vi "Add content to Engine library.vi"(6 "Project Name":string, 8 "error in":errorcluster, 9 "Project Root":path, 10 "CD Wizard - Internal Data":T1, 11 "CD Template":refnum<class "NIVS_PPL_Inline HW Interface.lvclass">) -> (0 "error out":errorcluster)   [LabVIEW 2020, in "NIVS_PPL_Inline HW Interface.lvclass"]
doc: "Add all virtual folders and VIs to the Engine library."
uses:
  NIVS_PPL_Inline HW Interface.lvclass
  NIVS_Consolidated_CDW_MetaDataObj/Internal data.ctl
  C:/dev/Karthick/FPGA Addons Packages/niveristand-custom-device-wizard/ProjectTemplate/Source/NI VeriStand/Custom Device/Template Classes/NIVS_CD Template/NIVS_CD Template.lvclass
  NIVS_Consolidated_CDW_MetaDataObj/CD Engine lvlib.ctl
  NIVS_Consolidated_CDW_MetaDataObj/Add Item - Type.ctl
  NIVS_CD Template/NIVS_CD Template.lvclass/NIVS_CD Template.ctl
  NIVS_Consolidated_CDW_MetaDataObj/CD Engine lvlib.vi
  NIVS_Consolidated_CDW_MetaDataObj/NIVS_Consolidated_CDW_MetaDataObj.lvclass
  NIVS_CD Template/NIVS_CD Template.lvclass
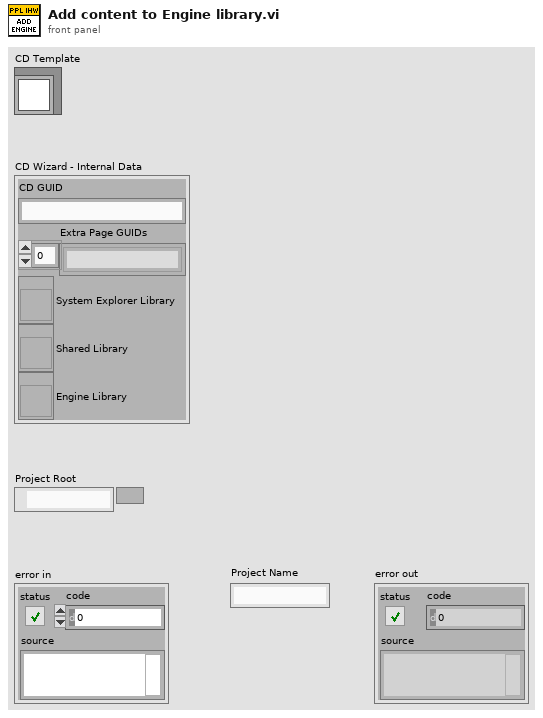
[diagram p1: front panel]
types:
  T1 = typedef "NIVS_Consolidated_CDW_MetaDataObj.lvclass/Internal data.ctl" = cluster{"CD GUID":string, "Extra Page GUIDs":string[], "System Explorer Library":refnum<vi>, "Shared Library":refnum<vi>, "Engine Library":refnum<vi>}
  T2 = typedef "NIVS_Consolidated_CDW_MetaDataObj.lvclass/CD Engine lvlib.ctl" = enum16{"LibraryFileName", "LibraryFolderName", "Engine.FolderName", "Engine.Init.FolderName", "Engine.Run.FolderName", "Engine.Shutdown.FolderName", "Types.FolderName", "Engine.RT Driver VI.TemplatePath", "Engine.RT Driver VI.FileName", "Engine.PPL.RT Driver VI_InlineAsync.FileName", "Engine.RTStateVariables.Name", "Engine.PPL.RTStateVariables.Name", "Engine.RTStateVariables.Name.NoExtension", "Engine.Async.NameExtension", "Engine.Async.TemplateName", "Engine.PPL.Async.TemplateName", "Engine.PPL.Async.InitVSGlobals.Name", "Engine.PPL.RT Driver VI_Inline.FileName", "Engine.LaunchCommandLoop.Name", "Engine.CommandLoop.Name"}
  T3 = typedef "NIVS_Consolidated_CDW_MetaDataObj.lvclass/Add Item - Type.ctl" = string
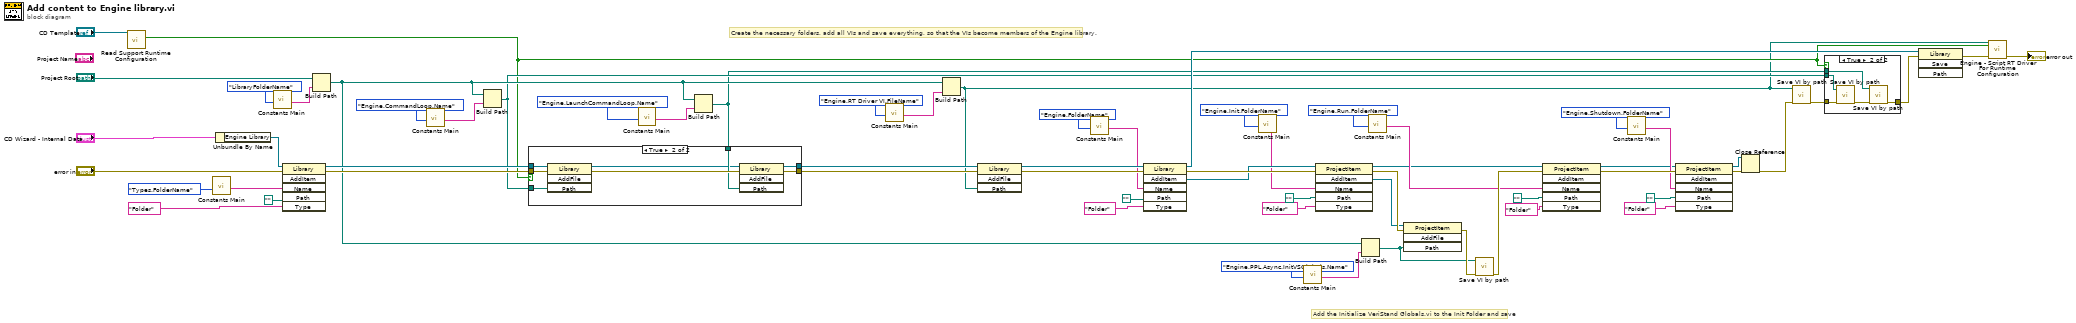
[diagram p0: block diagram]
diagram:
  # "Add the Initialize VeriStand Globals.vi to the Init Folder and save"
  # "Create the necessary folders, add all VIs and save everything, so that the VIs become members of the Engine library."
  n1 = call "Read Support Runtime Configuration.vi"("NIVS_CD Template in"="CD Template") -> ("Support Runtime Configuration"=w2:bool)  [unwired: 8 in, 2 out]
  n2 = call-poly "Constants Main.vi"("Action"=CD_Engine_lvlib."Types.FolderName") -> ("Output"=w17:string)  [unwired: 10 in]
  n3 = Unbundle By Name("CD Wizard - Internal Data") -> ("Engine Library"=w26:refnum<vi>)
  n4 = call-poly "Constants Main.vi"("Action"=CD_Engine_lvlib."LibraryFolderName") -> ("Output"=w24:string)  [unwired: 10 in]
  n5 = invoke class="Library" method="AddItem"(reference=w26, error in="error in", "Name"=w17, "Path"=path "", "Type"=T3 "Folder" ("Add Item - Type")) -> (reference out=w9:refnum<vi>, error out=w55:errorcluster)  [unwired: 1 in, 4 out]
  n6 = Build Path(base path="Project Root", name or relative path=w24) -> (appended path=w6:path)
  n7 = call-poly "Constants Main.vi"("Action"=CD_Engine_lvlib."Engine.CommandLoop.Name") -> ("Output"=w11:string)  [unwired: 10 in]
  n8 = Build Path(base path=w6, name or relative path=w11) -> (appended path=w4:path)
  n9 = call-poly "Constants Main.vi"("Action"=CD_Engine_lvlib."Engine.LaunchCommandLoop.Name") -> ("Output"=w7:string)  [unwired: 10 in]
  n10 = Build Path(base path=w6, name or relative path=w7) -> (appended path=w3:path)
  n11 = case shown="True" w2 {
    tunnel: w9 -> [w65 w71]
    tunnel: w55 -> [w66 w74]
    tunnel: w4 -> [_ w70]
    tunnel: w3 -> [_ w69]
    tunnel: [w65 w67] -> w5
    tunnel: [w66 w72] -> w54
    frame False {
    }
    frame True {
      n12 = invoke class="Library" method="AddFile"(reference=w71, error in=w74, "Path"=w70) -> (reference out=w68:refnum<vi>, error out=w73:errorcluster)  [unwired: 1 in, 2 out]
      n13 = invoke class="Library" method="AddFile"(reference=w68, error in=w73, "Path"=w69) -> (reference out=w67:refnum<vi>, error out=w72:errorcluster)  [unwired: 1 in, 2 out]
    }
  }
  n14 = call-poly "Constants Main.vi"("Action"=CD_Engine_lvlib."Engine.RT Driver VI.FileName") -> ("Output"=w22:string)  [unwired: 10 in]
  n15 = Build Path(base path=w6, name or relative path=w22) -> (appended path=w1:path)
  n16 = invoke class="Library" method="AddFile"(reference=w5, error in=w54, "Path"=w1) -> (reference out=w31:refnum<vi>, error out=w62:errorcluster)  [unwired: 1 in, 2 out]
  n17 = call-poly "Constants Main.vi"("Action"=CD_Engine_lvlib."Engine.FolderName") -> ("Output"=w29:string)  [unwired: 10 in]
  n18 = invoke class="Library" method="AddItem"(reference=w31, error in=w62, "Name"=w29, "Path"=path "", "Type"=T3 "Folder" ("Add Item - Type")) -> (reference out=w43:refnum<vi>, error out=w63:errorcluster, "AddItem"=w32:refnum<vi>)  [unwired: 1 in, 3 out]
  n19 = call-poly "Constants Main.vi"("Action"=CD_Engine_lvlib."Engine.Init.FolderName") -> ("Output"=w21:string)  [unwired: 10 in]
  n20 = call-poly "Constants Main.vi"("Action"=CD_Engine_lvlib."Engine.PPL.Async.InitVSGlobals.Name") -> ("Output"=w47:string)  [unwired: 10 in]
  n21 = invoke class="ProjectItem" method="AddItem"(reference=w32, error in=w63, "Name"=w21, "Path"=path "", "Type"=T3 "Folder" ("Add Item - Type")) -> (reference out=w34:refnum<vi>, error out=w64:errorcluster, "AddItem"=w48:refnum<vi>)  [unwired: 1 in, 3 out]
  n22 = Build Path(base path=w6, name or relative path=w47) -> (appended path=w49:path)
  n23 = call-poly "Constants Main.vi"("Action"=CD_Engine_lvlib."Engine.Run.FolderName") -> ("Output"=w36:string)  [unwired: 10 in]
  n24 = invoke class="ProjectItem" method="AddFile"(reference=w48, error in=w64, "Path"=w49) -> (error out=w57:errorcluster)  [unwired: 1 in, 3 out]
  n25 = call "Save VI by path.vi"("error in (no error)"=w57, "VI path"=w49) -> ("error out"=w56:errorcluster)  [unwired: 9 in]
  n26 = invoke class="ProjectItem" method="AddItem"(reference=w34, error in=w56, "Name"=w36, "Path"=path "", "Type"=T3 "Folder" ("Add Item - Type")) -> (reference out=w42:refnum<vi>, error out=w61:errorcluster)  [unwired: 1 in, 4 out]
  n27 = call-poly "Constants Main.vi"("Action"=CD_Engine_lvlib."Engine.Shutdown.FolderName") -> ("Output"=w44:string)  [unwired: 10 in]
  n28 = invoke class="ProjectItem" method="AddItem"(reference=w42, error in=w61, "Name"=w44, "Path"=path "", "Type"=T3 "Folder" ("Add Item - Type")) -> (reference out=w45:refnum<vi>, error out=w59:errorcluster)  [unwired: 1 in, 4 out]
  n29 = Close Reference(reference=w45, error in (no error)=w59) -> (error out=w60:errorcluster)
  n30 = call "Save VI by path.vi"("error in (no error)"=w60, "VI path"=w1) -> ("error out"=w53:errorcluster)  [unwired: 9 in]
  n31 = case shown="True" w2 {
    tunnel: w53 -> [w75 w80]
    tunnel: [w75 w78] -> w52
    tunnel: w4 -> [_ w77]
    tunnel: w3 -> [_ w76]
    frame False {
    }
    frame True {
      n32 = call "Save VI by path.vi"("error in (no error)"=w80, "VI path"=w77) -> ("error out"=w79:errorcluster)  [unwired: 9 in]
      n33 = call "Save VI by path.vi"("error in (no error)"=w79, "VI path"=w76) -> ("error out"=w78:errorcluster)  [unwired: 9 in]
    }
  }
  n34 = invoke class="Library" method="Save"(reference=w43, error in=w52) -> (error out=w51:errorcluster)  [unwired: 2 in, 3 out]
  n35 = call "Engine - Script RT Driver For Runtime Configuration.vi"("error in"=w51, "Support Runtime Configuration"=w2, "RT Driver VI Path"=w1) -> ("error out"=→"error out":errorcluster)  [unwired: 8 in]
